vi "Pt taches.vi"() -> ()   [LabVIEW 2022 SP3]
uses:
  Variables globales/Variable glob Pt.vi
panel:
  out "sortie d'erreur":errorcluster
  out "error out":errorcluster
  # "Lancement des tâches Pt100 pour chaque tâche définie"
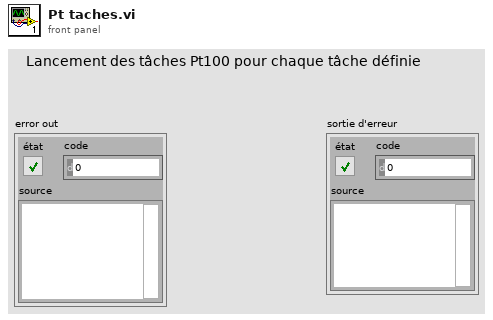
[diagram p1: front panel]
types:
  T1 = cluster{"Nom tache Pt":refnum<k21>, "Noms des Pt":string[], "Nb Pt":i16, "Selection Pt":bool[], "Nom Pt selectionnees":string[]}[]
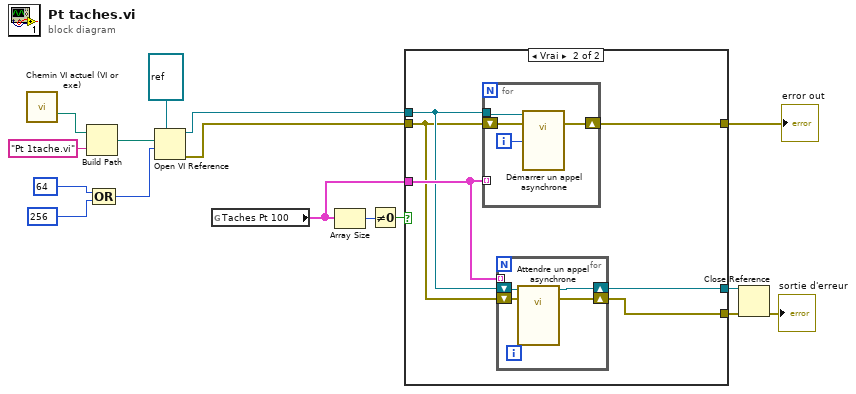
[diagram p0: block diagram]
diagram:
  n1 = call "Chemin VI actuel (VI or exe).vi"() -> ("VI or executable installation directory"=w3:path)  [unwired: 14 in, 1 out]
  n2 = Build Path(base path=w3, name or relative path="Pt 1tache.vi" ("nom ou chemin relatif")) -> (appended path=w16:path)
  n3 = Compound Arithmetic op=OR(64 ("options"), 256 ("options")) -> (w12:i32)
  n4 = Open VI Reference(type specifier VI Refnum (for type only)=refnum<vi> refnum ("spécificateur de type du refnum de VI (pour type seulement)"), vi path=w16, options=w12) -> (vi reference=w11:refnum<vi>, error out=w10:errorcluster)  [unwired: 3 in]
  n5 = global read "Variable glob Pt.vi" "Taches Pt 100"() -> (w2:T1)
  n6 = Array Size(array=w2) -> (size(s)=w5:i32)
  n7 = Not Equal To 0?(x=w5) -> (x != 0?=w4:bool)
  n8 = case shown="Vrai" w4 {
    tunnel: w11 -> [w17 w20]
    tunnel: w10 -> [w18 w19]
    tunnel: [w18 w24] -> w9
    tunnel: [w17 w23] -> w8
    tunnel: [w18 w22] -> w7
    tunnel: w2 -> [_ w21]
    frame False {
    }
    frame True {
      n9 = for {
        tunnel: w21 -> [_] mode=indexing
        tunnel: w20 -> [w29]
        shift-right: [w30] -> w24
        shift-left: w19 -> [w31]
        i -> [w32]
        n10 = call-by-ref "Démarrer un appel asynchrone"(reference=w29, error in=w31, "Indice tache"=w32) -> (error out=w30:errorcluster)  [unwired: 2 in, 2 out]
      }
      n11 = for {
        tunnel: w21 -> [_] mode=indexing
        shift-right: [w28] -> w23
        shift-left: w20 -> [w25]
        shift-right: [w26] -> w22
        shift-left: w19 -> [w27]
        n12 = call-by-ref "Attendre un appel asynchrone"(reference=w25, error in=w27) -> (reference out=w28:refnum<vi>, error out=w26:errorcluster)  [unwired: 3 in, 1 out]
      }
    }
  }
  "error out" <- w9
  n13 = Close Reference(reference=w8, error in (no error)=w7) -> (error out=→"sortie d'erreur":errorcluster)
